vi "Set LabVIEW Version.vi"(8 "error in":errorcluster, 11 "result json":string) -> (0 "error out":errorcluster, 3 "result json out":string)   [LabVIEW 2020, in "MCP Server.lvlib"]
doc: "Sets serverInfo.additionalDetails.labviewVersion of the initialize result to the version of the LabVIEW that runs the server.\n\nThe value is the application property Version Number as LabVIEW reports it, for example 26.3f0 for LabVIEW 2026 Q3 (major.minor, then f and the patch level). In a built application it is the version of the LabVIEW Run-Time Engine."
uses:
  MCP Server.lvlib
  58a92dd1-0b3c-4063-ade8-96245b9ef757.vi
  <vilib>/JDP Science/JSONtext/Variant to JSON Text.vi
  <vilib>/JDP Science/JSONtext/LVClass Serializer/JSONtext LVClass Serializer.lvclass
  <vilib>/JDP Science/JSONtext/JSONtext.lvlib
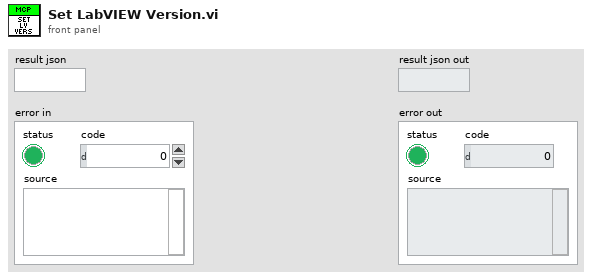
[diagram p1: front panel]
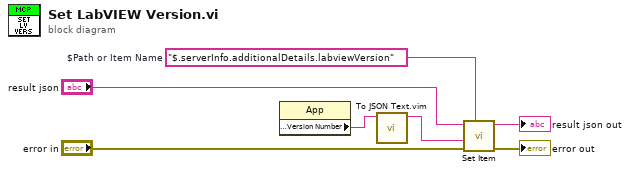
[diagram p0: block diagram]
diagram:
  w5 = "$.serverInfo.additionalDetails.labviewVersion"  # $Path or Item Name
  n1 = property class="App"() -> ("Application:Version Number"=w7:string)  [unwired: 2 in, 2 out]
  n2 = call "To JSON Text.vim"("Anything"=w7) -> ("<JSON>"=w4:string)  [unwired: 9 in, 1 out]
  n3 = call <vilib>:"Set Item.vi"("$Path or Item Name"=w5, "error in (no error)"="error in", "JSON to Insert"=w4, "JSON"="result json") -> ("error out"=→"error out":errorcluster, "<JSON>"=→"result json out":string)  [unwired: 4 in, 1 out]
